vi "Native_SetControlVIType.vi"() -> ()   [LabVIEW 2024]
panel:
  out "error out":errorcluster caption="错误输出"
  in  "control_vi_type":u32=2
  in  "target_path":path
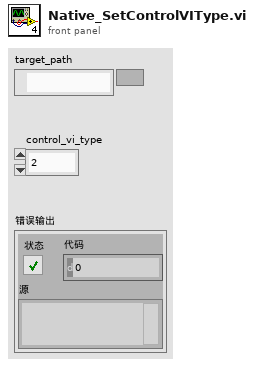
[diagram p1: front panel]
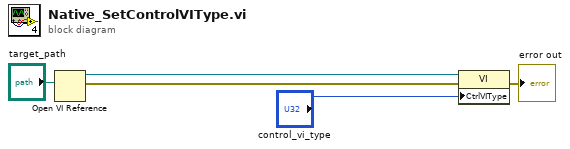
[diagram p0: block diagram]
diagram:
  n1 = Open VI Reference ("打开VI引用")(vi path="target_path") -> (vi reference=w4:refnum<vi>, error out=w2:errorcluster)  [unwired: 5 in]
  n2 = property on="属性节点" class="VI"(reference=w4, error in=w2, "CtrlVIType"="control_vi_type") -> (error out=→"error out":errorcluster)  [unwired: 1 out]
